vi "synchronize_mnu_with_directory.vi"(8 "error in (no error)":errorcluster, 9 "Synchronized Directory":path, 10 "MNU File":path, 11 "PackageFile in":refnum<class "PackageFile.lvclass">) -> (0 "error out":errorcluster, 3 "PackageFile out":refnum<class "PackageFile.lvclass">)   [LabVIEW 2020, in "vi_package_building_extensions.lvlib" / "PackageFile.lvclass"]
uses:
  PackageFile.lvclass
  PackageFile.lvclass/PackageFile.ctl
  vi_package_building_extensions.lvlib
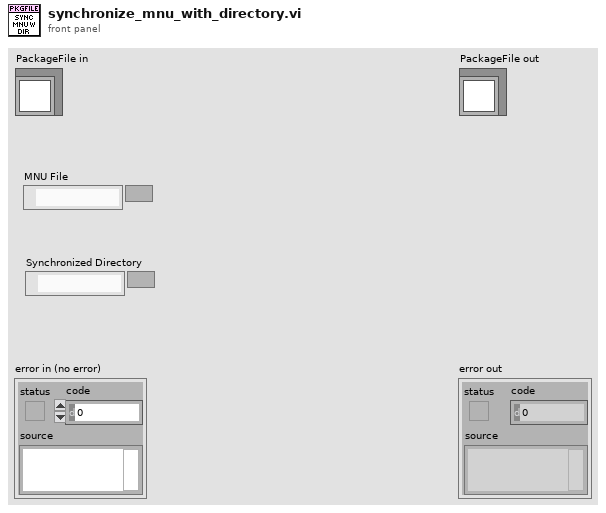
[diagram p1: front panel]
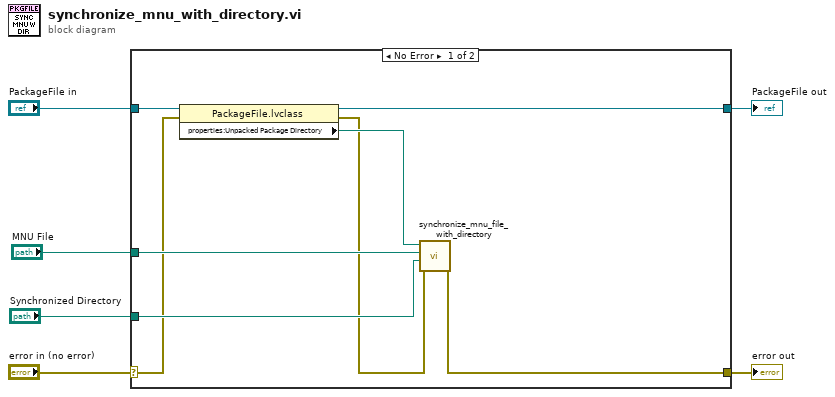
[diagram p0: block diagram]
diagram:
  n1 = case shown="No Error" "error in (no error)" {
    selector: "error in (no error)" -> [w8 w16]
    tunnel: [w13 w16] -> w5
    tunnel: [w10 w15] -> w3
    tunnel: "PackageFile in" -> [w14 w15]
    tunnel: "Synchronized Directory" -> [w12 _]
    tunnel: "MNU File" -> [w11 _]
    frame No Error {
      n2 = property class="PackageFile.lvclass"(reference=w14, error in=w8) -> (reference out=w10:refnum<class "PackageFile.lvclass">, error out=w7:errorcluster, "properties:Unpacked Package Directory"=w9:path)
      n3 = call "synchronize_mnu_file_with_directory.vi"("error in (no error)"=w7, "Synchronized Directory"=w12, "MNU File"=w11, "Unpacked Package Directory"=w9) -> ("error out"=w13:errorcluster)  [unwired: 7 in]
    }
    frame Error {
    }
  }
  "error out" <- w5
  "PackageFile out" <- w3
